vi "set LTE Modulation.vi"(8 "error in (no error)":errorcluster, 10 "Modulation":T1, 11 "Anritsu Call Box_Implement in":refnum<class "Anritsu Call Box_Implement.lvclass">) -> (0 "error out":errorcluster, 3 "Anritsu Call Box_Implement out":refnum<class "Anritsu Call Box_Implement.lvclass">)   [LabVIEW 2023, in "ANRITSU Call Box.lvlib" / "Anritsu Call Box_Implement.lvclass"]
uses:
  Anritsu Call Box_Implement.lvclass
  Anritsu Call Box_Implement.lvclass/Anritsu Call Box_Implement.ctl
  LTE/LTE.lvclass
  Type Definition/LTE Modulation Type.ctl
  ANRITSU Call Box.lvlib
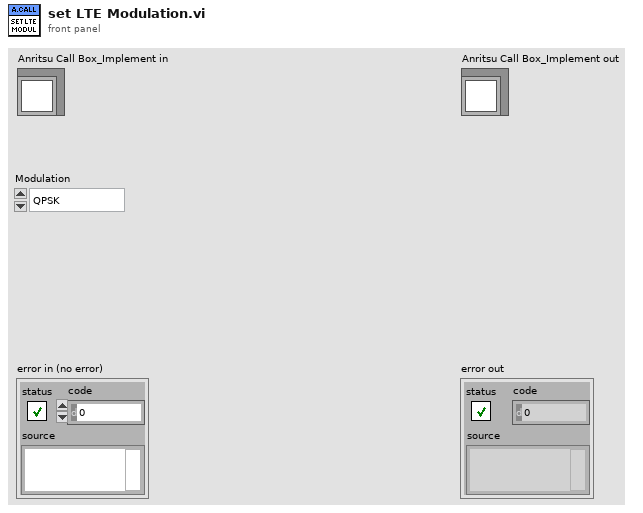
[diagram p1: front panel]
types:
  T1 = typedef "ANRITSU Call Box.lvlib/LTE Modulation Type.ctl" = enum16{"QPSK", "16QAM", "64QAM", "256QAM"}
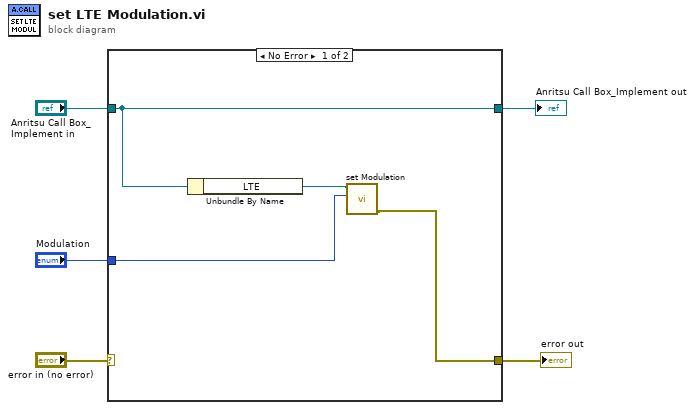
[diagram p0: block diagram]
diagram:
  n1 = case shown="No Error" "error in (no error)" {
    selector: "error in (no error)" -> [_ w10]
    tunnel: "Anritsu Call Box_Implement in" -> [w9 w11]
    tunnel: [w9 w11] -> w4
    tunnel: [w7 w10] -> w2
    tunnel: "Modulation" -> [w6 _]
    frame No Error {
      n2 = Unbundle By Name(w9) -> ("LTE"=w8:refnum<class "LTE.lvclass">)
      n3 = call "set Modulation.vi"("Modulation"=w6, "LTE in"=w8) -> ("error out"=w7:errorcluster)  [unwired: 8 in, 1 out]
    }
    frame Error {
    }
  }
  "error out" <- w2
  "Anritsu Call Box_Implement out" <- w4
